vi "ArmControlManager.vi"(0 "Arm Rotate Manual Control":dbl, 1 "Arm Extend Manual Control":dbl, 2 "rotate sensor unit conversion (ticks/rad)":dbl, 3 "extend sensor unit coversion (ticks/in)":dbl, 4 "Arm Rotate Motion Profile":T1[](array[typedef]) {"Time (ms)" items=["TrajectoryDuration_0ms"=0, "TrajectoryDuration_5ms"=5, "TrajectoryDuration_10ms"=10, "TrajectoryDuration_20ms"=20, "TrajectoryDuration_30ms"=30, "TrajectoryDuration_40ms"=40, "TrajectoryDuration_50ms"=50, "TrajectoryDuration_100ms"=100]}, 5 "Arm Extend Motion Profile":T1[](array[typedef]) {"Time (ms)" items=["TrajectoryDuration_0ms"=0, "TrajectoryDuration_5ms"=5, "TrajectoryDuration_10ms"=10, "TrajectoryDuration_20ms"=20, "TrajectoryDuration_30ms"=30, "TrajectoryDuration_40ms"=40, "TrajectoryDuration_50ms"=50, "TrajectoryDuration_100ms"=100]}, 6 "ArmCompleteNotifier":refnum<notifier>, 8 "Arm Extend Motor DevRef":T4={"DeviceStatus"={"status"=FALSE, "code"=0, "source"=""}, "Type"=enum."PWM", "PWM"={"PWM Channel"=enum."PWM 1", "DeadBand"={"Name"="", "maxPositivePwm"=0, "minPositivePwm"=0, "centerPwm"=0, "maxNegativePwm"=0, "minNegativePwm"=0, "angularRange"=0}}, "CAN"={"Device Number"=0, "SetOutput VI Ref"=variant(enum8{"Percent VBus", "Current", "Speed", "Position", "Voltage"} enum."Percent VBus"), "GetOutput VI Ref"=variant(refnum<k1> refnum), "Enable VI Ref"=variant(dbl 12.0), "Disable VI Ref"=variant(enum8{"Percent VBus", "Speed", "Position", "Slave", "Unchanged / Invalid", "Voltage Compensation", "Current", "Motion Profile"} enum."Percent VBus"), "Data"=variant}, "Invert"=FALSE, "DIO PWM"={"PWM \"Enable\" Channel"=enum."Invalid", "DIOChannel"=enum."Invalid", "PWM Rate"=0.0}}, 9 "New Motion Profile":bool, 10 "Arm Rotate Motor DevRef":T4={"DeviceStatus"={"status"=FALSE, "code"=0, "source"=""}, "Type"=enum."PWM", "PWM"={"PWM Channel"=enum."PWM 1", "DeadBand"={"Name"="", "maxPositivePwm"=0, "minPositivePwm"=0, "centerPwm"=0, "maxNegativePwm"=0, "minNegativePwm"=0, "angularRange"=0}}, "CAN"={"Device Number"=0, "SetOutput VI Ref"=variant(enum8{"Percent VBus", "Current", "Speed", "Position", "Voltage"} enum."Percent VBus"), "GetOutput VI Ref"=variant(refnum<k1> refnum), "Enable VI Ref"=variant(dbl 12.0), "Disable VI Ref"=variant(enum8{"Percent VBus", "Speed", "Position", "Slave", "Unchanged / Invalid", "Voltage Compensation", "Current", "Motion Profile"} enum."Percent VBus"), "Data"=variant}, "Invert"=FALSE, "DIO PWM"={"PWM \"Enable\" Channel"=enum."Invalid", "DIOChannel"=enum."Invalid", "PWM Rate"=0.0}}) -> (14 "Arm Control State":T3)   [LabVIEW 2017]
uses:
  General/MotionProfiling/TypeDefs/TrajectoryPoint.ctl
  <vilib>/Rock Robotics/WPI/ThirdParty/Phoenix-LabVIEW/Motor Controller/Controls/CTRE_Phoenix_MotorControl_TrajectoryPointTimeDur.ctl
  General/MotionProfiling/TypeDefs/MotionProfileControlState.ctl
  <vilib>/Rock Robotics/WPI/MotorControl/WPI_MotorControlDeviceRef.ctl
  <vilib>/Rock Robotics/WPI/MotorControl/WPI_MotorControlType.ctl
  <vilib>/Rock Robotics/SystemInterfaces/DIO/FPGA_DIOPWMChannel.ctl
  <vilib>/Rock Robotics/WPI/PWM/WPI_PWMDeadband.ctl
  <vilib>/Rock Robotics/SystemInterfaces/DIO/FPGA_DIOChannel.ctl
  General/MotionProfiling/TypeDefs/MPSendState.ctl
  <vilib>/Rock Robotics/WPI/DriverStation/WPI_DriverStationRobotMode2.ctl
  ArgosLib/Signal Processing/TypeDefs/EdgeDetector_Type.ctl
  <vilib>/Rock Robotics/WPI/ThirdParty/Phoenix-LabVIEW/Motor Controller/Controls/CTRE_Phoenix_MotorControl_ControlMode.ctl
  Global_Var-RefNum/MotionProfileControlData.vi
  <vilib>/Rock Robotics/WPI/ThirdParty/Phoenix-LabVIEW/Motor Controller/Get/CTRE_Phoenix_MotorController_GetSelectedSensorData.vi
  <vilib>/Rock Robotics/WPI/ThirdParty/Phoenix-LabVIEW/Motor Controller/Get/CTRE_Phoenix_MotorController_GetVoltage.vi
  Global_Var-RefNum/LEDData.vi
  ArgosLib/ArgosLib.lvlib
panel:
  in  "MP State Timeout (ms)":u32
  in  "Tab Control":enum32{"I/O", "Calibration", "Status"}(tab)
  in  "ExtendErrorThresh (in)":dbl=3.0
  in  "RotateErrorThresh (rad)":dbl=0.1745
  in  "ClearMotionProfile":bool
  in  "StallDetectTime(ms)":u32=200
  in  "EnableStallDetection":bool
  out "Max Extend Speed (Sensor Units per 100 ms)":i32
  out "Max Rotate Speed (Sensor Units per 100 ms)":i32
  in  "Reset Rotate Max":bool
  in  "Reset Extend Max":bool
  in  "Reset Extend Sensor":bool
  in  "Reset Rotate Sensor":bool
  in  "Extend Position (in)":dbl=-44.0
  in  "Rotate Position (rad)":dbl=1.57
  out "MP Send State":T9
  out "Rotate":T10
  out "Extension":T10
  out "Rotate":T11
  out "Extension":T11
  out "ExtendFaults":T12
  out "RotateFaults":T12
  out "Arm Tracking":cluster{dbl[], dbl[]}[](graph)
  out "ArmRotateV":dbl(graph)
  out "ArmExtensionV":dbl(graph)
  out "ArmExtension":T11(graph)
  out "ArmRotation":T11(graph)
  # "10 degrees or 3 inches\nerror for 200ms will\ncancel motion"
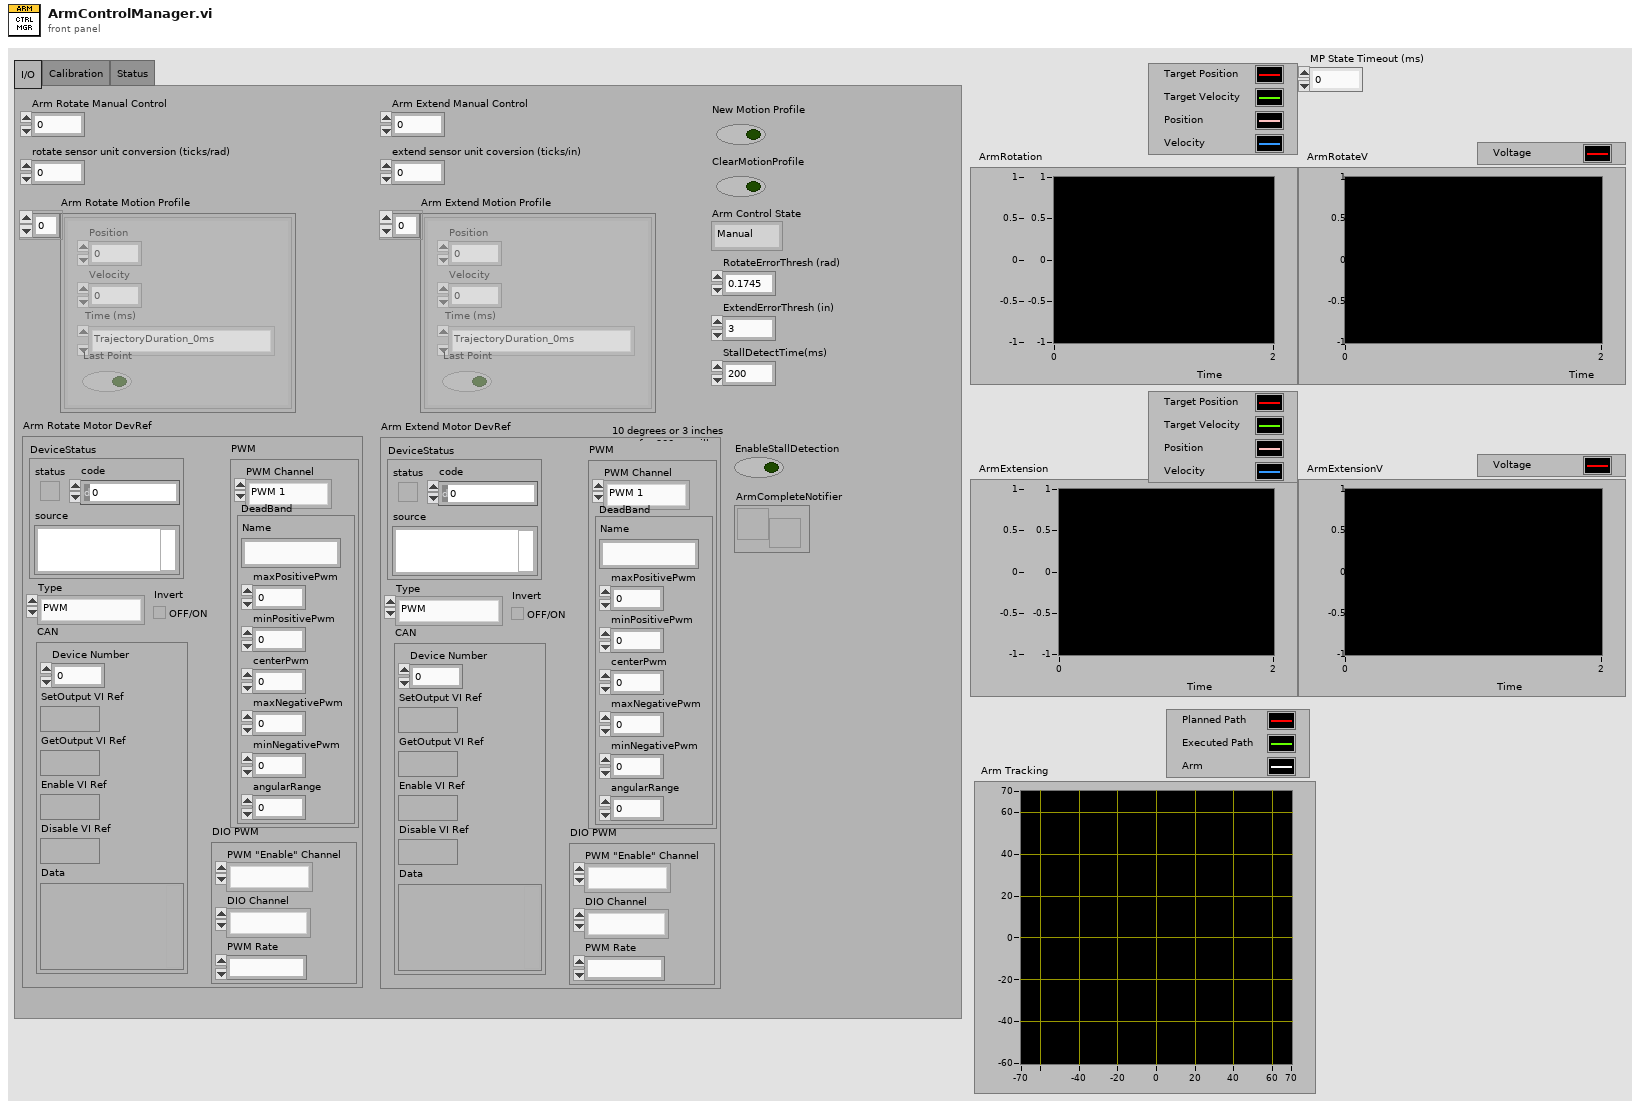
[diagram p1: front panel]
types:
  T1 = typedef "TrajectoryPoint.ctl" = cluster{"Position ":dbl, "Velocity ":dbl, "Time (ms)":T2, "Last Point":bool}
  T2 = typedef "CTRE_Phoenix_MotorControl_TrajectoryPointTimeDur.ctl" = i32
  T3 = typedef "MotionProfileControlState.ctl" = enum16{"Manual", "Auto_Idle", "Auto_Run"}
  T4 = typedef "WPI_MotorControlDeviceRef.ctl" = cluster{"DeviceStatus":errorcluster, "Type":T5, "PWM":cluster{"PWM Channel":T6, "DeadBand":T7}, "CAN":cluster{"Device Number":u8, "SetOutput VI Ref":variant, "GetOutput VI Ref":variant, "Enable VI Ref":variant, "Disable VI Ref":variant, "Data":variant}, "Invert":bool, "DIO PWM":cluster{"PWM \"Enable\" Channel":T6, "DIOChannel":T8, "PWM Rate":dbl}}
  T5 = typedef "WPI_MotorControlType.ctl" = enum16{"PWM", "CAN", "DIO PWM"}
  T6 = typedef "FPGA_DIOPWMChannel.ctl" = enum8{"PWM 0", "PWM 1", "PWM 2", "PWM 3", "PWM 4", "PWM 5", "PWM 6", "PWM 7", "PWM 8", "PWM 9", "PWM MXP 0", "PWM MXP 1", "PWM MXP 2", "PWM MXP 3", "PWM MXP 4", "PWM MXP 5", "PWM MXP 6", "PWM MXP 7", "PWM MXP 8", "PWM MXP 9", "Invalid"}
  T7 = typedef "WPI_PWMDeadband.ctl" = cluster{"Name":string, "maxPositivePwm":i32, "minPositivePwm":i32, "centerPwm":i32, "maxNegativePwm":i32, "minNegativePwm":i32, "angularRange":u16}
  T8 = typedef "FPGA_DIOChannel.ctl" = enum8{"DIO 0", "DIO 1", "DIO 2", "DIO 3", "DIO 4", "DIO 5", "DIO 6", "DIO 7", "DIO 8", "DIO 9", "DIO MXP 0", "DIO MXP 1", "DIO MXP 2", "DIO MXP 3", "DIO MXP 4", "DIO MXP 5", "DIO MXP 6", "DIO MXP 7", "DIO MXP 8", "DIO MXP 9", "DIO MXP 10", "DIO MXP 11", "DIO MXP 12", "DIO MXP 13", "DIO MXP 14", "DIO MXP 15", "SPI Port CS1", "SPI Port CS2", "SPI Port CS3", "SPI Port MISO", "SPI Port MOSI", "Invalid"}
  T9 = typedef "MPSendState.ctl" = enum16{"Disable", "Commit Points", "Enable", "Done", "Failed"}
  T10 = cluster{"Top Buffer Remaining":i32, "Top Buffer Count":i32, "Bottom Buffer Count":i32, "Has Underrun?":bool, "Is Underrun?":bool, "Active Point Valid?":bool, "Is Last?":bool, "Profile Slot Select 0":i32, "Output Enable":i32, "Time Duration (ms)":i32, "Profile Slot Select 1":i32}
  T11 = cluster{"Position (Sensor Units)":i32, "Velocity (Sensor Units per 100 ms)":i32, "Position (Raw Sensor Units)":i32, "Velocity (Raw Sensor Units per 100 ms)":i32}
  T12 = cluster{"Under Voltage":bool, "Forward Limit Switch":bool, "Reverse Limit Switch":bool, "Forward Soft Limit":bool, "Reverse Soft Limit":bool, "Hardware Failure":bool, "Reset During Enable":bool, "Sensor Overflow":bool, "Sensor Out of Phase":bool, "Hardware ESD Reset":bool, "Remote Loss of Signal":bool}
  T13 = typedef "WPI_DriverStationRobotMode2.ctl" = enum16{"Autonomous Disabled", "Autonomous Enabled", "Teleop Disabled", "Teleop Enabled", "Disconnected", "Finish", "Test Disabled", "Test Enabled", "Emergency Stopped"}
  T14 = typedef "ArgosLib.lvlib/EdgeDetector_Type.ctl" = enum16{"RisingEdge", "FallingEdge", "Both"}
  T15 = cluster{"Position (Sensor Units)":i32, "Velocity (Sensor Units per 100 ms)":i32, "Position (Raw Sensor Units)":i32, "Velocity (Raw Sensor Units per 100 ms)":i32}[]
  T16 = typedef "CTRE_Phoenix_MotorControl_ControlMode.ctl" = u16
  T17 = typedef "ArmMotionProfileControl.ctl" = cluster{"ControlMutex":T18, "Trajectory Points":T1[], "CurrentIndex":u32}
  T18 = typedef "Semaphore RefNum" = refnum<k1>
  T19 = cluster{"Position (Sensor Units)":i32, "Velocity (Sensor Units per 100 ms)":i32, "Position (Raw Sensor Units)":i32, i32}
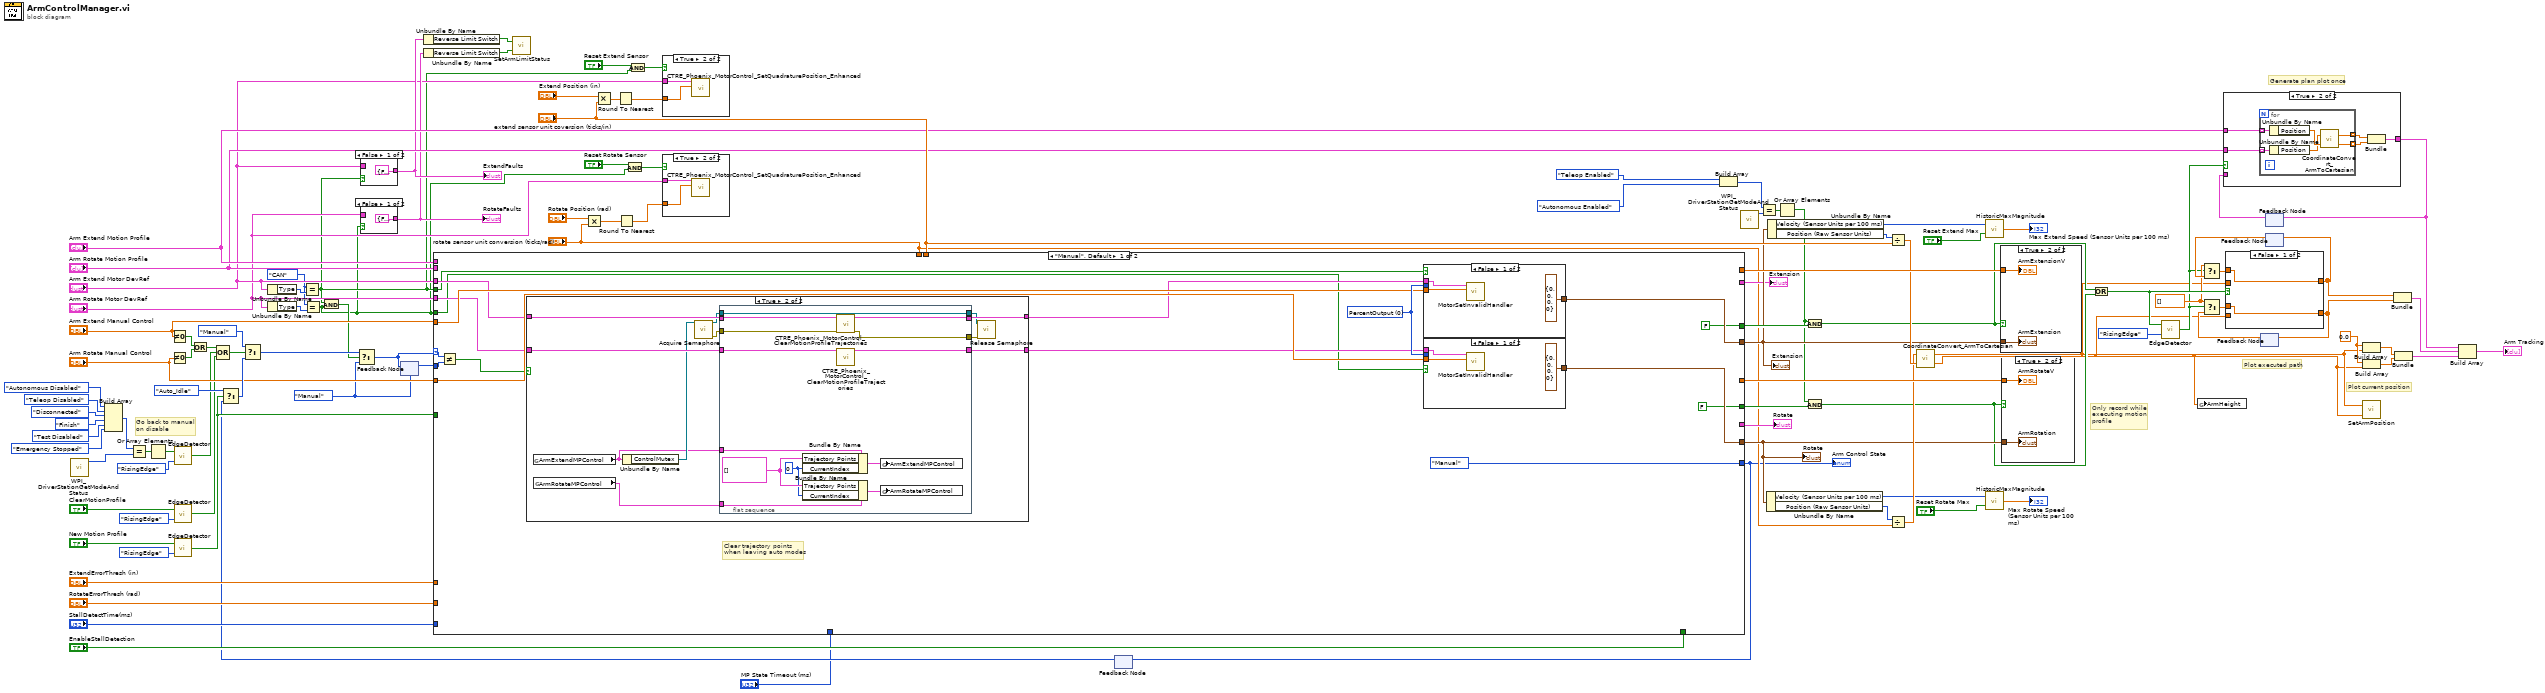
[diagram p0: block diagram]
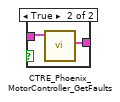
[diagram p2: hidden frame]
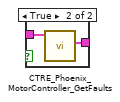
[diagram p3: hidden frame]
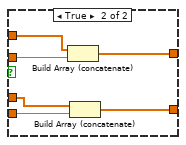
[diagram p5: hidden frame]
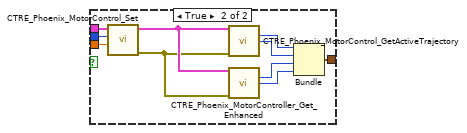
[diagram p10: hidden frame]
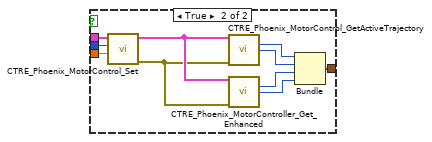
[diagram p11: hidden frame]
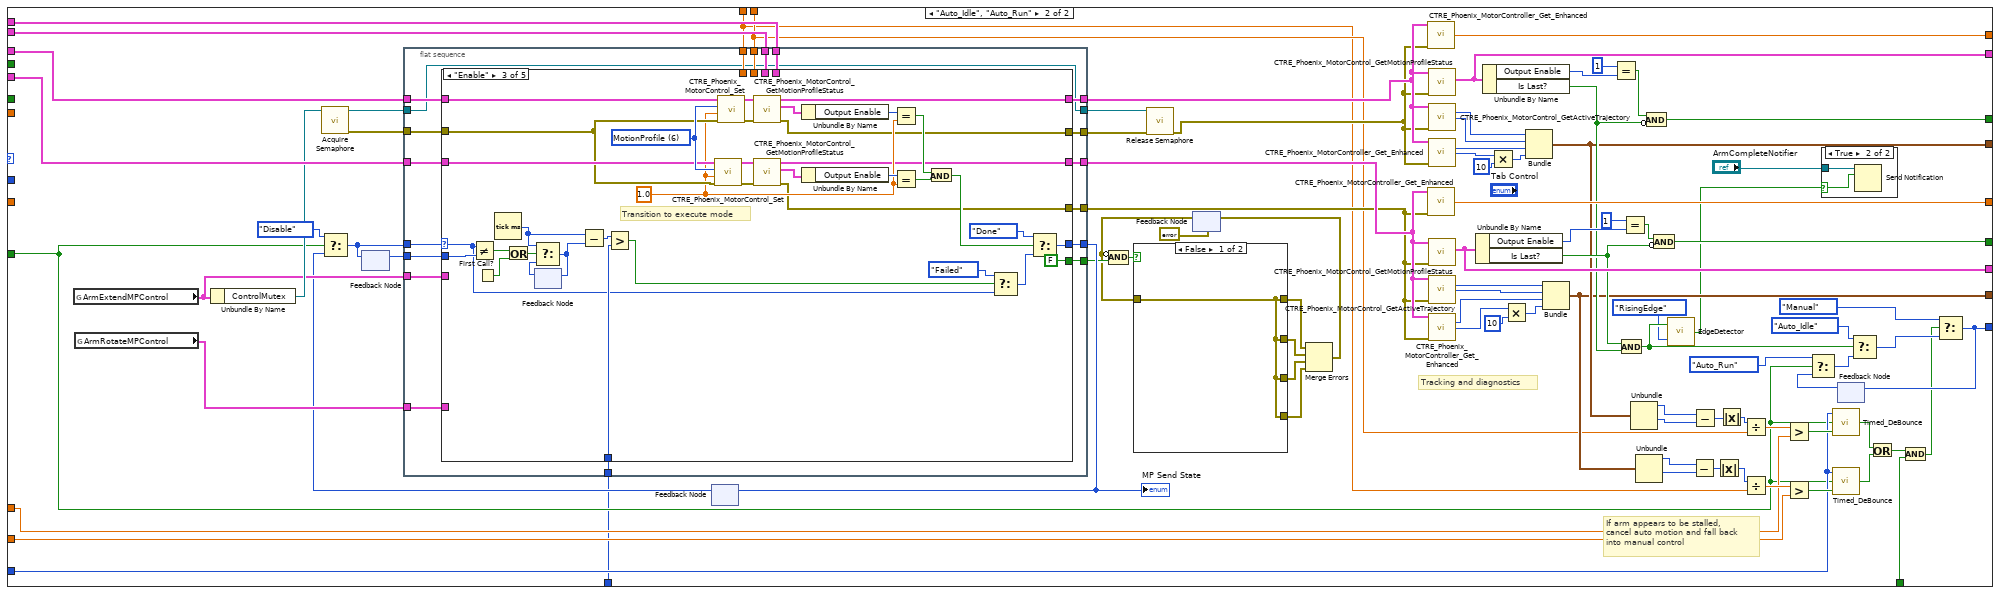
[diagram p13: hidden frame]
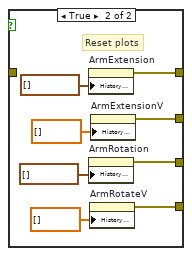
[diagram p15: hidden frame]
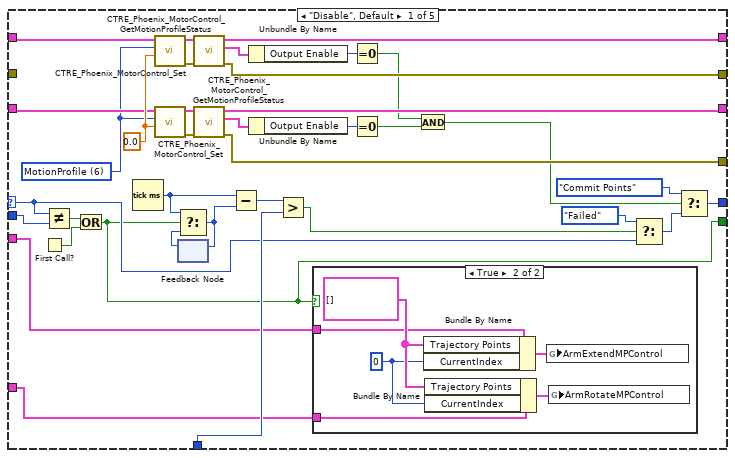
[diagram p16: hidden frame]
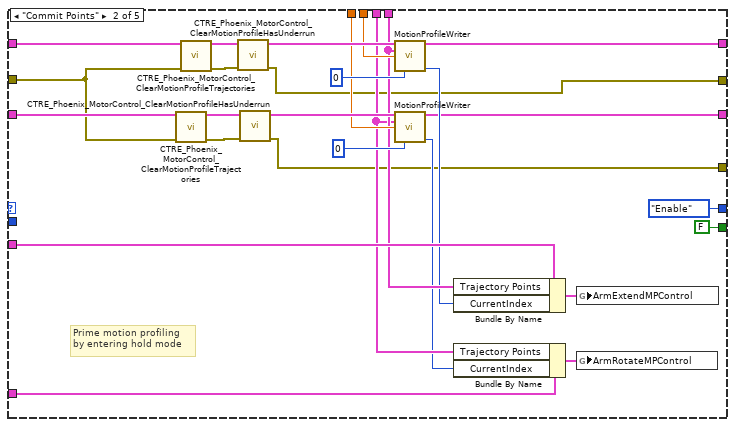
[diagram p18: hidden frame]
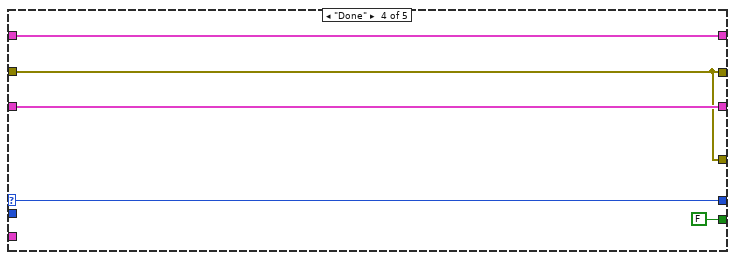
[diagram p19: hidden frame]
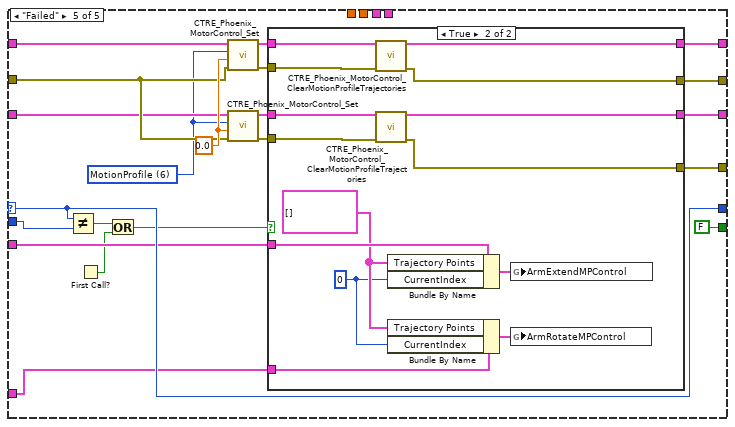
[diagram p20: hidden frame]
diagram:
  w7 = MotionProfileControlState."Manual" ("t")
  w10 = WPI_MotorControlType."CAN" ("x")
  w40 = dbl[] [] ("t")
  w74 = 0.0 ("element")
  # "Plot current position"
  # "Plot executed path"
  # "Generate plan plot once"
  # "Go back to manual\non disable"
  # "Only record while\nexecuting motion\nprofile"
  n1 = call <vilib>:"WPI_DriverStationGetModeAndStatus.vi"() -> ("Robot Mode"=w66:T13)  [unwired: 10 in, 1 out]
  n2 = Build Array(WPI_DriverStationRobotMode2."Autonomous Disabled" ("Robot Mode"), WPI_DriverStationRobotMode2."Teleop Disabled" ("Robot Mode"), WPI_DriverStationRobotMode2."Disconnected" ("Robot Mode"), WPI_DriverStationRobotMode2."Finish" ("Robot Mode"), WPI_DriverStationRobotMode2."Test Disabled" ("Robot Mode"), WPI_DriverStationRobotMode2."Emergency Stopped" ("Robot Mode")) -> (w67:T13[])
  n3 = Equal?(x=w67, y=w66) -> (x = y?=w65:bool[])
  n4 = Or Array Elements(Boolean array=w65) -> (logical OR=w64:bool)
  n5 = Not Equal To 0?(x="Arm Extend Manual Control") -> (x != 0?=w110:bool)
  n6 = Not Equal To 0?(x="Arm Rotate Manual Control") -> (x != 0?=w109:bool)
  n7 = call "EdgeDetector.vi"("DetectorType"=EdgeDetector_Type."RisingEdge", "Input"=w64) -> ("Edge"=w61:bool)
  n8 = call "EdgeDetector.vi"("DetectorType"=EdgeDetector_Type."RisingEdge", "Input"="ClearMotionProfile") -> ("Edge"=w62:bool)
  n9 = call "EdgeDetector.vi"("DetectorType"=EdgeDetector_Type."RisingEdge", "Input"="New Motion Profile") -> ("Edge"=w103:bool)
  n10 = Or(x=w110, y=w109) -> (x .or. y?=w92:bool)
  n11 = Compound Arithmetic op=OR(w92, w61, w62) -> (w93:bool)
  n12 = Unbundle By Name("Arm Extend Motor DevRef") -> ("Type"=w12:T5)
  n13 = Unbundle By Name("Arm Rotate Motor DevRef") -> ("Type"=w11:T5)
  n14 = Equal?(x=w10, y=w12) -> (x = y?=w2:bool)
  n15 = Equal?(x=w10, y=w11) -> (x = y?=w1:bool)
  n16 = And(x=w2, y=w1) -> (x .and. y?=w6:bool)
  n17 = case shown="False" w2 {
    tunnel: [T12 {"Under Voltage"=FALSE, "Forward Limit Switch"=FALSE, "Reverse Limit Switch"=FALSE, "Forward Soft Limit"=FALSE, "Reverse Soft Limit"=FALSE, "Hardware Failure"=FALSE, "Reset During Enable"=FALSE, "Sensor Overflow"=FALSE, "Sensor Out of Phase"=FALSE, "Hardware ESD Reset"=FALSE, "Remote Loss of Signal"=FALSE} ("Faults") w113] -> w18
    tunnel: "Arm Extend Motor DevRef" -> [_ w112]
    frame False {
    }
    frame True {
      n18 = call <vilib>:"CTRE_Phoenix_MotorController_GetFaults.vi"("PhoenixMotorControlDevRef"=w112) -> ("Faults"=w113:T12)  [unwired: 8 in, 2 out]
    }
  }
  "ExtendFaults" <- w18
  n19 = case shown="False" w1 {
    tunnel: [T12 {"Under Voltage"=FALSE, "Forward Limit Switch"=FALSE, "Reverse Limit Switch"=FALSE, "Forward Soft Limit"=FALSE, "Reverse Soft Limit"=FALSE, "Hardware Failure"=FALSE, "Reset During Enable"=FALSE, "Sensor Overflow"=FALSE, "Sensor Out of Phase"=FALSE, "Hardware ESD Reset"=FALSE, "Remote Loss of Signal"=FALSE} ("Faults") w116] -> w17
    tunnel: "Arm Rotate Motor DevRef" -> [_ w115]
    frame False {
    }
    frame True {
      n20 = call <vilib>:"CTRE_Phoenix_MotorController_GetFaults.vi"("PhoenixMotorControlDevRef"=w115) -> ("Faults"=w116:T12)  [unwired: 8 in, 2 out]
    }
  }
  "RotateFaults" <- w17
  n21 = feedback #1(w7) -> (w23:T3)
  n22 = Unbundle By Name(w18) -> ("Reverse Limit Switch"=w16:bool)
  n23 = Unbundle By Name(w17) -> ("Reverse Limit Switch"=w15:bool)
  n24 = call "SetArmLimitStatus.vi"("ArmRotateLimit"=w15, "ArmExtendLimit"=w16) -> ()  [unwired: 1 in]
  n25 = Multiply(x="Rotate Position (rad)", y="rotate sensor unit conversion (ticks/rad)") -> (x*y=w78:dbl)
  n26 = Multiply(x="Extend Position (in)", y="extend sensor unit coversion (ticks/in)") -> (x*y=w81:dbl)
  n27 = Round To Nearest(number=w81) -> (nearest integer value=w80:dbl)
  n28 = Round To Nearest(number=w78) -> (nearest integer value=w77:dbl)
  n29 = And(x="Reset Rotate Sensor", y=w1) -> (x .and. y?=w4:bool)
  n30 = And(x="Reset Extend Sensor", y=w2) -> (x .and. y?=w5:bool)
  n31 = case shown="True" w5 {
    tunnel: "Arm Extend Motor DevRef" -> [_ w118]
    tunnel: w80 -> [_ w117]
    frame False {
    }
    frame True {
      n32 = call <vilib>:"CTRE_Phoenix_MotorControl_SetQuadraturePosition_Enhanced.vi"("New Position"=w117, "PhoenixMotorControlDevRef"=w118) -> ()  [unwired: 8 in, 2 out]
    }
  }
  n33 = case shown="True" w4 {
    tunnel: "Arm Rotate Motor DevRef" -> [_ w120]
    tunnel: w77 -> [_ w119]
    frame False {
    }
    frame True {
      n34 = call <vilib>:"CTRE_Phoenix_MotorControl_SetQuadraturePosition_Enhanced.vi"("New Position"=w119, "PhoenixMotorControlDevRef"=w120) -> ()  [unwired: 8 in, 2 out]
    }
  }
  n35 = feedback #2() -> (w22:T3)  [unwired: 1 in]
  n36 = Select(t=MotionProfileControlState."Auto_Idle", s=w103, f=w22) -> (s? t:f=w107:T3)
  n37 = Select(t=MotionProfileControlState."Manual" ("Arm Control State"), s=w93, f=w107) -> (s? t:f=w9:T3)
  n38 = Select(t=w9, s=w6, f=w7) -> (s? t:f=w8:T3)
  n39 = feedback-in #1(w8) -> ()
  n40 = case shown="\"Manual\", Default" w8 {
    selector: w8 -> [w135 _]
    tunnel: "Arm Extend Motor DevRef" -> [w127 w239]
    tunnel: "Arm Rotate Motor DevRef" -> [w126 w238]
    tunnel: "Arm Extend Manual Control" -> [w128 _]
    tunnel: "Arm Rotate Manual Control" -> [w136 _]
    tunnel: w23 -> [w134 _]
    tunnel: w103 -> [_ w209]
    tunnel: "Arm Extend Motion Profile" -> [_ w241]
    tunnel: "Arm Rotate Motion Profile" -> [_ w240]
    tunnel: [MotionProfileControlState."Manual" ("Arm Control State") w244] -> w24
    tunnel: [w132 w229] -> w76
    tunnel: [w131 w228] -> w75
    tunnel: [FALSE w271] -> w96
    tunnel: [FALSE w267] -> w98
    tunnel: [_ w260] -> w95
    tunnel: [_ w259] -> w94
    tunnel: "extend sensor unit coversion (ticks/in)" -> [_ w219]
    tunnel: "rotate sensor unit conversion (ticks/rad)" -> [_ w217]
    tunnel: [_ w255] -> w54
    tunnel: [_ w254] -> w53
    tunnel: "ExtendErrorThresh (in)" -> [_ w250]
    tunnel: "RotateErrorThresh (rad)" -> [_ w251]
    tunnel: "StallDetectTime(ms)" -> [_ w247]
    tunnel: "EnableStallDetection" -> [_ w221]
    tunnel: "MP State Timeout (ms)" -> [_ w204]
    tunnel: w2 -> [w122 _]
    tunnel: w1 -> [w121 _]
    frame "Manual", Default {
      w137 = T16 0 items=["PercentOutput"=0, "Position"=1, "Velocity"=2, "Current"=3, "Follower"=5, "MotionProfile"=6, "MotionMagic"=7, "MotionMagicArc"=8, "MotionProfileArc"=10, "Disabled"=15] ("Control Mode")
      # "Clear trajectory points\nwhen leaving auto modes"
      n41 = Not Equal?(x=w135, y=w134) -> (x != y?=w123:bool)
      n42 = case shown="True" w123 {
        tunnel: w127 -> [w165 w176]
        tunnel: [w165 w175] -> w125
        tunnel: w126 -> [w164 w174]
        tunnel: [w164 w173] -> w124
        frame False {
        }
        frame True {
          n43 = global read "MotionProfileControlData.vi" "ArmExtendMPControl"() -> (w169:T17)
          n44 = global read "MotionProfileControlData.vi" "ArmRotateMPControl"() -> (w168:T17)
          n45 = Unbundle By Name(w169) -> ("ControlMutex"=w171:T18)
          n46 = call <vilib>:"Acquire Semaphore.vi"("semaphore"=w171) -> ("error out"=w172:errorcluster, "semaphore out"=w167:T18)  [unwired: 4 in, 1 out]
          n47 = flat-sequence {
            tunnel: w176 -> [w189]
            tunnel: [w188] -> w175
            tunnel: w174 -> [w187]
            tunnel: [w186] -> w173
            tunnel: w172 -> [w185]
            tunnel: [w184] -> w170
            tunnel: w169 -> [w183]
            tunnel: w168 -> [w182]
            tunnel: w167 -> [w177]
            tunnel: [w177] -> w166
            frame #0 {
              w180 = u32 0 ("CurrentIndex")
              w181 = T1[] [] ("Trajectory Points")
              n48 = Bundle By Name(cluster=w183, "Trajectory Points"=w181, "CurrentIndex"=w180) -> (w178:T17)
              n49 = Bundle By Name(cluster=w182, "Trajectory Points"=w181, "CurrentIndex"=w180) -> (w179:T17)
              n50 = call <vilib>:"CTRE_Phoenix_MotorControl_ClearMotionProfileTrajectories.vi"("PhoenixMotorControlDevRef"=w189, "error in"=w185) -> ("PhoenixMotorControlDevRef"=w188:T4, "error out"=w184:errorcluster)  [unwired: 12 in]
              n51 = call <vilib>:"CTRE_Phoenix_MotorControl_ClearMotionProfileTrajectories.vi"("PhoenixMotorControlDevRef"=w187) -> ("PhoenixMotorControlDevRef"=w186:T4)  [unwired: 13 in, 1 out]
              n52 = global write "MotionProfileControlData.vi" "ArmExtendMPControl"(w178) -> ()
              n53 = global write "MotionProfileControlData.vi" "ArmRotateMPControl"(w179) -> ()
            }
          }
          n54 = call <vilib>:"Release Semaphore.vi"("error in (no error)"=w170, "semaphore"=w166) -> ()  [unwired: 4 in, 2 out]
        }
      }
      n55 = case shown="False" w122 {
        tunnel: w137 -> [_ w163]
        tunnel: [T11 {"Position (Sensor Units)"=0, "Velocity (Sensor Units per 100 ms)"=0, "Position (Raw Sensor Units)"=0, "Velocity (Raw Sensor Units per 100 ms)"=0} w162] -> w132
        tunnel: w128 -> [w152 w155]
        tunnel: w125 -> [w153 w154]
        frame False {
          n56 = call "MotorSetInvalidHandler.vi"("Output"=w152, "MotorControlDevRef"=w153) -> ()  [unwired: 7 in, 3 out]
        }
        frame True {
          n57 = call <vilib>:"CTRE_Phoenix_MotorControl_Set.vi"("Output"=w155, "Control Mode"=w163, "PhoenixMotorControlDevRef"=w154) -> ("error out"=w160:errorcluster, "PhoenixMotorControlDevRef"=w161:T4)  [unwired: 7 in]
          n58 = call <vilib>:"CTRE_Phoenix_MotorControl_GetActiveTrajectory.vi"("PhoenixMotorControlDevRef"=w161, "error in"=w160) -> ("Position (Sensor Units)"=w159:i32, "Velocity (Sensor Units per 100 ms)"=w158:i32)  [unwired: 9 in, 3 out]
          n59 = call-poly <vilib>:"CTRE_Phoenix_MotorController_Get_Enhanced.vi"("PhoenixMotorControlDevRef"=w161, "error in"=w160) -> ("Position (Raw Sensor Units)"=w157:i32, "Velocity (Raw Sensor Units per 100 ms)"=w156:i32)  [unwired: 10 in, 2 out]
          n60 = Bundle("Position (Sensor Units)"=w159, "Velocity (Sensor Units per 100 ms)"=w158, "Position (Raw Sensor Units)"=w157, "Velocity (Raw Sensor Units per 100 ms)"=w156) -> (w162:T11)  [unwired: 1 in]
        }
      }
      n61 = case shown="False" w121 {
        tunnel: w137 -> [_ w150]
        tunnel: w136 -> [w139 w149]
        tunnel: [T11 {"Position (Sensor Units)"=0, "Velocity (Sensor Units per 100 ms)"=0, "Position (Raw Sensor Units)"=0, "Velocity (Raw Sensor Units per 100 ms)"=0} w142] -> w131
        tunnel: w124 -> [w140 w141]
        frame False {
          n62 = call "MotorSetInvalidHandler.vi"("Output"=w139, "MotorControlDevRef"=w140) -> ()  [unwired: 7 in, 3 out]
        }
        frame True {
          n63 = call <vilib>:"CTRE_Phoenix_MotorControl_Set.vi"("Output"=w149, "Control Mode"=w150, "PhoenixMotorControlDevRef"=w141) -> ("error out"=w147:errorcluster, "PhoenixMotorControlDevRef"=w148:T4)  [unwired: 7 in]
          n64 = call <vilib>:"CTRE_Phoenix_MotorControl_GetActiveTrajectory.vi"("PhoenixMotorControlDevRef"=w148, "error in"=w147) -> ("Position (Sensor Units)"=w146:i32, "Velocity (Sensor Units per 100 ms)"=w145:i32)  [unwired: 9 in, 3 out]
          n65 = call-poly <vilib>:"CTRE_Phoenix_MotorController_Get_Enhanced.vi"("PhoenixMotorControlDevRef"=w148, "error in"=w147) -> ("Position (Raw Sensor Units)"=w144:i32, "Velocity (Raw Sensor Units per 100 ms)"=w143:i32)  [unwired: 10 in, 2 out]
          n66 = Bundle("Position (Sensor Units)"=w146, "Velocity (Sensor Units per 100 ms)"=w145, "Position (Raw Sensor Units)"=w144, "Velocity (Raw Sensor Units per 100 ms)"=w143) -> (w142:T11)  [unwired: 1 in]
        }
      }
    }
    frame "Auto_Idle", "Auto_Run" {
      # "If arm appears to be stalled,\ncancel auto motion and fall back\ninto manual control"
      # "Tracking and diagnostics"
      n67 = global read "MotionProfileControlData.vi" "ArmExtendMPControl"() -> (w214:T17)
      n68 = global read "MotionProfileControlData.vi" "ArmRotateMPControl"() -> (w213:T17)
      n69 = Unbundle By Name(w214) -> ("ControlMutex"=w215:T18)
      n70 = call <vilib>:"Acquire Semaphore.vi"("semaphore"=w215) -> ("error out"=w216:errorcluster, "semaphore out"=w211:T18)  [unwired: 4 in, 1 out]
      n71 = feedback #3() -> (w205:T9)  [unwired: 1 in]
      n72 = flat-sequence {
        tunnel: w239 -> [w311]
        tunnel: w238 -> [w310]
        tunnel: w216 -> [w309]
        tunnel: w219 -> [w308]
        tunnel: w217 -> [w307]
        tunnel: [w306] -> w237
        tunnel: [w305] -> w235
        tunnel: w214 -> [w304]
        tunnel: w213 -> [w303]
        tunnel: w241 -> [w302]
        tunnel: w240 -> [w301]
        tunnel: [w300] -> w212
        tunnel: [w299] -> w234
        tunnel: w211 -> [w298]
        tunnel: [w298] -> w210
        tunnel: w206 -> [w297]
        tunnel: [w296] -> w203
        tunnel: w205 -> [w295]
        tunnel: w204 -> [w294]
        tunnel: [w293] -> w193
        frame #0 {
          n73 = case shown="\"Enable\"" w297 {
            selector: w297 -> [w315 _ w385 w418 w437]
            tunnel: w311 -> [w342 w362 w415 w421 w441]
            tunnel: w310 -> [w341 w361 w414 w420 w439]
            tunnel: w309 -> [_ w360 w413 w419 w440]
            tunnel: w308 -> [_ w372 _ _ _]
            tunnel: w307 -> [_ w371 _ _ _]
            tunnel: [w334 w358 w389 w421 w430] -> w306
            tunnel: [w335 w359 w387 w420 w428] -> w305
            tunnel: w304 -> [w318 w370 _ _ w425]
            tunnel: w303 -> [w317 w369 _ _ w426]
            tunnel: w302 -> [_ w368 _ _ _]
            tunnel: w301 -> [_ w367 _ _ _]
            tunnel: [w333 w356 w388 w419 w429] -> w300
            tunnel: [w332 w357 w386 w419 w427] -> w299
            tunnel: [w325 MPSendState."Enable" ("MP Send State") w403 w418 w437] -> w296
            tunnel: w295 -> [w324 _ w408 _ w436]
            tunnel: w294 -> [w319 _ w407 _ _]
            tunnel: [w313 FALSE FALSE FALSE FALSE] -> w293
            frame "Disable", Default {
              w347 = 0.0 ("Output")
              w340 = T16 6 items=["PercentOutput"=0, "Position"=1, "Velocity"=2, "Current"=3, "Follower"=5, "MotionProfile"=6, "MotionMagic"=7, "MotionMagicArc"=8, "MotionProfileArc"=10, "Disabled"=15] ("Control Mode")
              n74 = First Call?() -> (First Call?: T/F=w312:bool)
              n75 = Not Equal?(x=w315, y=w324) -> (x != y?=w314:bool)
              n76 = Or(x=w314, y=w312) -> (x .or. y?=w313:bool)
              n77 = Tick Count (ms)() -> (millisecond timer value=w322:u32)
              n78 = call <vilib>:"CTRE_Phoenix_MotorControl_Set.vi"("Output"=w347, "Control Mode"=w340, "PhoenixMotorControlDevRef"=w342) -> ("error out"=w345:errorcluster, "PhoenixMotorControlDevRef"=w346:T4)  [unwired: 7 in]
              n79 = call <vilib>:"CTRE_Phoenix_MotorControl_Set.vi"("Output"=w347, "Control Mode"=w340, "PhoenixMotorControlDevRef"=w341) -> ("error out"=w344:errorcluster, "PhoenixMotorControlDevRef"=w343:T4)  [unwired: 7 in]
              n80 = feedback #4() -> (w323:u32)  [unwired: 1 in]
              n81 = Select(t=w322, s=w313, f=w323) -> (s? t:f=w321:u32)
              n82 = feedback-in #4(w321) -> ()
              n83 = call <vilib>:"CTRE_Phoenix_MotorControl_GetMotionProfileStatus.vi"("error in"=w345, "PhoenixMotorControlDevRef"=w346) -> ("error out"=w333:errorcluster, "Motion Profile Status"=w339:T10, "PhoenixMotorControlDevRef"=w334:T4)  [unwired: 7 in]
              n84 = call <vilib>:"CTRE_Phoenix_MotorControl_GetMotionProfileStatus.vi"("error in"=w344, "PhoenixMotorControlDevRef"=w343) -> ("error out"=w332:errorcluster, "Motion Profile Status"=w338:T10, "PhoenixMotorControlDevRef"=w335:T4)  [unwired: 7 in]
              n85 = Subtract(x=w322, y=w321) -> (x-y=w320:u32)
              n86 = Unbundle By Name(w339) -> ("Output Enable"=w337:i32)
              n87 = Unbundle By Name(w338) -> ("Output Enable"=w336:i32)
              n88 = Greater?(x=w320, y=w319) -> (0:w316:bool)
              n89 = case shown="True" w313 {
                tunnel: w318 -> [_ w349]
                tunnel: w317 -> [_ w348]
                frame False {
                }
                frame True {
                  w350 = u32 0 ("CurrentIndex")
                  w351 = T1[] [] ("Trajectory Points")
                  n90 = Bundle By Name(cluster=w349, "Trajectory Points"=w351, "CurrentIndex"=w350) -> (w353:T17)
                  n91 = Bundle By Name(cluster=w348, "Trajectory Points"=w351, "CurrentIndex"=w350) -> (w352:T17)
                  n92 = global write "MotionProfileControlData.vi" "ArmExtendMPControl"(w353) -> ()
                  n93 = global write "MotionProfileControlData.vi" "ArmRotateMPControl"(w352) -> ()
                }
              }
              n94 = Equal To 0?(x=w337) -> (x = 0?=w331:bool)
              n95 = Equal To 0?(x=w336) -> (x = 0?=w330:bool)
              n96 = And(x=w331, y=w330) -> (x .and. y?=w329:bool)
              n97 = Select(t=MPSendState."Failed", s=w316, f=w315) -> (s? t:f=w328:T9)
              n98 = Select(t=MPSendState."Commit Points", s=w329, f=w328) -> (s? t:f=w325:T9)
            }
            frame "Commit Points" {
              # "Prime motion profiling\nby entering hold mode"
              n99 = call <vilib>:"CTRE_Phoenix_MotorControl_ClearMotionProfileTrajectories.vi"("PhoenixMotorControlDevRef"=w361, "error in"=w360) -> ("PhoenixMotorControlDevRef"=w380:T4, "error out"=w379:errorcluster)  [unwired: 12 in]
              n100 = call <vilib>:"CTRE_Phoenix_MotorControl_ClearMotionProfileTrajectories.vi"("PhoenixMotorControlDevRef"=w362, "error in"=w360) -> ("PhoenixMotorControlDevRef"=w378:T4, "error out"=w377:errorcluster)  [unwired: 12 in]
              n101 = call <vilib>:"CTRE_Phoenix_MotorControl_ClearMotionProfileHasUnderrun.vi"("error in"=w377, "PhoenixMotorControlDevRef"=w378) -> ("error out"=w356:errorcluster, "PhoenixMotorControlDevRef"=w376:T4)  [unwired: 8 in]
              n102 = call <vilib>:"CTRE_Phoenix_MotorControl_ClearMotionProfileHasUnderrun.vi"("error in"=w379, "PhoenixMotorControlDevRef"=w380) -> ("error out"=w357:errorcluster, "PhoenixMotorControlDevRef"=w375:T4)  [unwired: 8 in]
              n103 = call "MotionProfileWriter.vi"("PhoenixMotorControlDevRef"=w376, "Trajectory Points"=w368, "Sensor unit conversion"=w372, "startIndex"=0) -> ("PhoenixMotorControlDevRef Out"=w358:T4, "endIndex"=w366:i32)  [unwired: 10 in]
              n104 = call "MotionProfileWriter.vi"("PhoenixMotorControlDevRef"=w375, "Trajectory Points"=w367, "Sensor unit conversion"=w371, "startIndex"=0) -> ("PhoenixMotorControlDevRef Out"=w359:T4, "endIndex"=w365:i32)  [unwired: 10 in]
              n105 = Bundle By Name(cluster=w370, "Trajectory Points"=w368, "CurrentIndex"=w366) -> (w364:T17)
              n106 = Bundle By Name(cluster=w369, "Trajectory Points"=w367, "CurrentIndex"=w365) -> (w363:T17)
              n107 = global write "MotionProfileControlData.vi" "ArmExtendMPControl"(w364) -> ()
              n108 = global write "MotionProfileControlData.vi" "ArmRotateMPControl"(w363) -> ()
            }
            frame "Enable" {
              w391 = 1.0 ("Output")
              w416 = T16 6 items=["PercentOutput"=0, "Position"=1, "Velocity"=2, "Current"=3, "Follower"=5, "MotionProfile"=6, "MotionMagic"=7, "MotionMagicArc"=8, "MotionProfileArc"=10, "Disabled"=15] ("Control Mode")
              # "Transition to execute mode"
              n109 = Not Equal?(x=w385, y=w408) -> (x != y?=w382:bool)
              n110 = First Call?() -> (First Call?: T/F=w381:bool)
              n111 = Tick Count (ms)() -> (millisecond timer value=w411:u32)
              n112 = Or(x=w382, y=w381) -> (x .or. y?=w383:bool)
              n113 = feedback #5() -> (w412:u32)  [unwired: 1 in]
              n114 = Select(t=w411, s=w383, f=w412) -> (s? t:f=w410:u32)
              n115 = feedback-in #5(w410) -> ()
              n116 = Subtract(x=w411, y=w410) -> (x-y=w409:u32)
              n117 = Greater?(x=w409, y=w407) -> (0:w402:bool)
              n118 = call <vilib>:"CTRE_Phoenix_MotorControl_Set.vi"("error in (no error)"=w413, "Output"=w391, "Control Mode"=w416, "PhoenixMotorControlDevRef"=w414) -> ("error out"=w396:errorcluster, "PhoenixMotorControlDevRef"=w397:T4)  [unwired: 6 in]
              n119 = call <vilib>:"CTRE_Phoenix_MotorControl_Set.vi"("error in (no error)"=w413, "Output"=w391, "Control Mode"=w416, "PhoenixMotorControlDevRef"=w415) -> ("error out"=w394:errorcluster, "PhoenixMotorControlDevRef"=w395:T4)  [unwired: 6 in]
              n120 = call <vilib>:"CTRE_Phoenix_MotorControl_GetMotionProfileStatus.vi"("error in"=w394, "PhoenixMotorControlDevRef"=w395) -> ("error out"=w388:errorcluster, "Motion Profile Status"=w401:T10, "PhoenixMotorControlDevRef"=w389:T4)  [unwired: 7 in]
              n121 = call <vilib>:"CTRE_Phoenix_MotorControl_GetMotionProfileStatus.vi"("error in"=w396, "PhoenixMotorControlDevRef"=w397) -> ("error out"=w386:errorcluster, "Motion Profile Status"=w400:T10, "PhoenixMotorControlDevRef"=w387:T4)  [unwired: 7 in]
              n122 = Unbundle By Name(w401) -> ("Output Enable"=w393:i32)
              n123 = Unbundle By Name(w400) -> ("Output Enable"=w392:i32)
              n124 = Equal?(x=w393, y=w391) -> (x = y?=w399:bool)
              n125 = Equal?(x=w392, y=w391) -> (x = y?=w398:bool)
              n126 = And(x=w399, y=w398) -> (x .and. y?=w390:bool)
              n127 = Select(t=MPSendState."Failed", s=w402, f=w385) -> (s? t:f=w406:T9)
              n128 = Select(t=MPSendState."Done", s=w390, f=w406) -> (s? t:f=w403:T9)
            }
            frame "Done" {
            }
            frame "Failed" {
              w442 = 0.0 ("Output")
              w438 = T16 6 items=["PercentOutput"=0, "Position"=1, "Velocity"=2, "Current"=3, "Follower"=5, "MotionProfile"=6, "MotionMagic"=7, "MotionMagicArc"=8, "MotionProfileArc"=10, "Disabled"=15] ("Control Mode")
              n129 = Not Equal?(x=w437, y=w436) -> (x != y?=w435:bool)
              n130 = First Call?() -> (First Call?: T/F=w422:bool)
              n131 = Or(x=w435, y=w422) -> (x .or. y?=w423:bool)
              n132 = call <vilib>:"CTRE_Phoenix_MotorControl_Set.vi"("error in (no error)"=w440, "Output"=w442, "Control Mode"=w438, "PhoenixMotorControlDevRef"=w441) -> ("error out"=w432:errorcluster, "PhoenixMotorControlDevRef"=w434:T4)  [unwired: 6 in]
              n133 = call <vilib>:"CTRE_Phoenix_MotorControl_Set.vi"("error in (no error)"=w440, "Output"=w442, "Control Mode"=w438, "PhoenixMotorControlDevRef"=w439) -> ("error out"=w431:errorcluster, "PhoenixMotorControlDevRef"=w433:T4)  [unwired: 6 in]
              n134 = case shown="True" w423 {
                tunnel: w434 -> [w446 w460]
                tunnel: w433 -> [w444 w458]
                tunnel: w432 -> [w445 w459]
                tunnel: w431 -> [w443 w457]
                tunnel: [w446 w456] -> w430
                tunnel: [w445 w455] -> w429
                tunnel: [w444 w454] -> w428
                tunnel: [w443 w453] -> w427
                tunnel: w426 -> [_ w450]
                tunnel: w425 -> [_ w449]
                frame False {
                }
                frame True {
                  w447 = u32 0 ("CurrentIndex")
                  w448 = T1[] [] ("Trajectory Points")
                  n135 = call <vilib>:"CTRE_Phoenix_MotorControl_ClearMotionProfileTrajectories.vi"("PhoenixMotorControlDevRef"=w460, "error in"=w459) -> ("PhoenixMotorControlDevRef"=w456:T4, "error out"=w455:errorcluster)  [unwired: 12 in]
                  n136 = call <vilib>:"CTRE_Phoenix_MotorControl_ClearMotionProfileTrajectories.vi"("PhoenixMotorControlDevRef"=w458, "error in"=w457) -> ("PhoenixMotorControlDevRef"=w454:T4, "error out"=w453:errorcluster)  [unwired: 12 in]
                  n137 = Bundle By Name(cluster=w449, "Trajectory Points"=w448, "CurrentIndex"=w447) -> (w452:T17)
                  n138 = Bundle By Name(cluster=w450, "Trajectory Points"=w448, "CurrentIndex"=w447) -> (w451:T17)
                  n139 = global write "MotionProfileControlData.vi" "ArmExtendMPControl"(w452) -> ()
                  n140 = global write "MotionProfileControlData.vi" "ArmRotateMPControl"(w451) -> ()
                }
              }
            }
          }
        }
      }
      n141 = feedback-in #6(w203) -> ()
      n142 = feedback #6() -> (w207:T9)  [unwired: 1 in]
      n143 = Select(t=MPSendState."Disable" ("MP Send State"), s=w209, f=w207) -> (s? t:f=w206:T9)
      n144 = feedback-in #3(w206) -> ()
      n145 = call <vilib>:"Release Semaphore.vi"("error in (no error)"=w212, "semaphore"=w210) -> ("error out"=w236:errorcluster)  [unwired: 4 in, 1 out]
      n146 = feedback #7(errorcluster {"status"=FALSE, "code"=0, "source"=""} ("error IO")) -> (w190:errorcluster)
      n147 = Compound Arithmetic op=AND(invert w190, w193) -> (w192:bool)
      n148 = case shown="False" w192 {
        tunnel: [w284 w288] -> w198
        tunnel: [w284 w287] -> w197
        tunnel: [w284 w286] -> w196
        tunnel: [w284 w285] -> w195
        tunnel: w190 -> [w284 _]
        frame False {
        }
        frame True {
          # "Reset plots"
          n149 = property on="ArmExtension" class="WFChart (strict)"("History Data"=T15 []) -> (error out=w288:errorcluster)  [unwired: 2 in, 1 out]
          n150 = property on="ArmRotation" class="WFChart (strict)"("History Data"=T15 []) -> (error out=w286:errorcluster)  [unwired: 2 in, 1 out]
          n151 = property on="ArmRotateV" class="WFChart (strict)"("History Data"=dbl[] []) -> (error out=w285:errorcluster)  [unwired: 2 in, 1 out]
          n152 = property on="ArmExtensionV" class="WFChart (strict)"("History Data"=dbl[] []) -> (error out=w287:errorcluster)  [unwired: 2 in, 1 out]
        }
      }
      n153 = Merge Errors(w198, w197, w196, w195) -> (w194:errorcluster)
      n154 = feedback-in #7(w194) -> ()
      n155 = call-poly <vilib>:"CTRE_Phoenix_MotorController_Get_Enhanced.vi"("PhoenixMotorControlDevRef"=w237, "error in"=w236) -> ("Output Voltage"=w259:dbl)  [unwired: 9 in, 4 out]
      n156 = call-poly <vilib>:"CTRE_Phoenix_MotorController_Get_Enhanced.vi"("PhoenixMotorControlDevRef"=w235, "error in"=w234) -> ("Output Voltage"=w260:dbl)  [unwired: 9 in, 4 out]
      n157 = call <vilib>:"CTRE_Phoenix_MotorControl_GetMotionProfileStatus.vi"("error in"=w236, "PhoenixMotorControlDevRef"=w237) -> ("Motion Profile Status"=w254:T10)  [unwired: 7 in, 2 out]
      n158 = call <vilib>:"CTRE_Phoenix_MotorControl_GetActiveTrajectory.vi"("PhoenixMotorControlDevRef"=w237, "error in"=w236) -> ("Position (Sensor Units)"=w280:i32, "Velocity (Sensor Units per 100 ms)"=w279:i32)  [unwired: 9 in, 3 out]
      n159 = call-poly <vilib>:"CTRE_Phoenix_MotorController_Get_Enhanced.vi"("PhoenixMotorControlDevRef"=w237, "error in"=w236) -> ("Position (Raw Sensor Units)"=w278:i32, "Velocity (Raw Sensor Units per 100 ms)"=w262:i32)  [unwired: 10 in, 2 out]
      n160 = call <vilib>:"CTRE_Phoenix_MotorControl_GetMotionProfileStatus.vi"("error in"=w234, "PhoenixMotorControlDevRef"=w235) -> ("Motion Profile Status"=w255:T10)  [unwired: 7 in, 2 out]
      n161 = call <vilib>:"CTRE_Phoenix_MotorControl_GetActiveTrajectory.vi"("PhoenixMotorControlDevRef"=w235, "error in"=w234) -> ("Position (Sensor Units)"=w277:i32, "Velocity (Sensor Units per 100 ms)"=w276:i32)  [unwired: 9 in, 3 out]
      n162 = call-poly <vilib>:"CTRE_Phoenix_MotorController_Get_Enhanced.vi"("PhoenixMotorControlDevRef"=w235, "error in"=w234) -> ("Position (Raw Sensor Units)"=w275:i32, "Velocity (Raw Sensor Units per 100 ms)"=w265:i32)  [unwired: 10 in, 2 out]
      n163 = Unbundle By Name(w255) -> ("Output Enable"=w268:i32, "Is Last?"=w231:bool)
      n164 = Unbundle By Name(w254) -> ("Output Enable"=w274:i32, "Is Last?"=w230:bool)
      n165 = Multiply(x=w262, y=10) -> (x*y=w263:i32)
      n166 = Multiply(x=w265, y=10) -> (x*y=w266:i32)
      n167 = Bundle("Position (Sensor Units)"=w280, "Velocity (Sensor Units per 100 ms)"=w279, "Position (Raw Sensor Units)"=w278, w263) -> (w229:T19)  [unwired: 1 in]
      n168 = Bundle("Position (Sensor Units)"=w277, "Velocity (Sensor Units per 100 ms)"=w276, "Position (Raw Sensor Units)"=w275, w266) -> (w228:T19)  [unwired: 1 in]
      n169 = Equal?(x=1, y=w274) -> (x = y?=w272:bool)
      n170 = Equal?(x=1, y=w268) -> (x = y?=w270:bool)
      n171 = Compound Arithmetic op=AND(w231, w230) -> (w202:bool)
      n172 = Unbundle(w229) -> ("Position (Sensor Units)"=w227:i32, "Position (Raw Sensor Units)"=w226:i32)  [unwired: 2 out]
      n173 = Unbundle(w228) -> ("Position (Sensor Units)"=w225:i32, "Position (Raw Sensor Units)"=w224:i32)  [unwired: 2 out]
      n174 = Compound Arithmetic op=AND(w272, invert w230) -> (w271:bool)
      n175 = Compound Arithmetic op=AND(w270, invert w231) -> (w267:bool)
      n176 = call "EdgeDetector.vi"("DetectorType"=EdgeDetector_Type."RisingEdge", "Input"=w202) -> ("Edge"=w200:bool)
      n177 = Subtract(x=w225, y=w224) -> (x-y=w232:i32)
      n178 = Subtract(x=w227, y=w226) -> (x-y=w233:i32)
      n179 = Absolute Value(x=w232) -> (abs(x)=w218:i32)
      n180 = Absolute Value(x=w233) -> (abs(x)=w220:i32)
      n181 = Divide(x=w220, y=w219) -> (x/y=w253:dbl)
      n182 = Divide(x=w218, y=w217) -> (x/y=w252:dbl)
      n183 = Greater?(x=w253, y=w250) -> (0:w249:bool)
      n184 = Greater?(x=w252, y=w251) -> (0:w248:bool)
      n185 = case shown="True" w200 {
        selector: w200 -> [_ w283]
        tunnel: "ArmCompleteNotifier" -> [_ w282]
        frame False {
        }
        frame True {
          n186 = Send Notification(notification=w283, notifier=w282) -> ()  [unwired: 1 in, 2 out]
        }
      }
      n187 = call "Timed_DeBounce.vi"("Input"=w249, "Reset"=w209, "Hold Time(ms)"=w247) -> ("Output"=w246:bool)
      n188 = call "Timed_DeBounce.vi"("Input"=w248, "Reset"=w209, "Hold Time(ms)"=w247) -> ("Output"=w245:bool)
      n189 = feedback #8() -> (w256:T3)  [unwired: 1 in]
      n190 = Select(t=MotionProfileControlState."Auto_Run" ("Arm Control State"), s=w209, f=w256) -> (s? t:f=w257:T3)
      n191 = Select(t=MotionProfileControlState."Auto_Idle" ("Arm Control State"), s=w202, f=w257) -> (s? t:f=w243:T3)
      n192 = Or(x=w246, y=w245) -> (x .or. y?=w223:bool)
      n193 = And(x=w223, y=w221) -> (x .and. y?=w222:bool)
      n194 = Select(t=MotionProfileControlState."Manual", s=w222, f=w243) -> (s? t:f=w244:T3)
      n195 = feedback-in #8(w244) -> ()
      "MP Send State" <- w203
    }
  }
  "Arm Control State" <- w24
  "Extension" <- w76
  "Rotate" <- w75
  "Rotate" <- w54
  "Extension" <- w53
  n196 = feedback-in #2(w24) -> ()
  n197 = Build Array(WPI_DriverStationRobotMode2."Teleop Enabled" ("Robot Mode"), WPI_DriverStationRobotMode2."Autonomous Enabled" ("Robot Mode")) -> (w30:T13[])
  n198 = call <vilib>:"WPI_DriverStationGetModeAndStatus.vi"() -> ("Robot Mode"=w34:T13)  [unwired: 10 in, 1 out]
  n199 = Equal?(x=w30, y=w34) -> (x = y?=w33:bool[])
  n200 = Unbundle By Name(w75) -> ("Velocity (Sensor Units per 100 ms)"=w57:i32, "Position (Raw Sensor Units)"=w90:i32)
  n201 = Unbundle By Name(w76) -> ("Velocity (Sensor Units per 100 ms)"=w60:i32, "Position (Raw Sensor Units)"=w91:i32)
  n202 = Or Array Elements(Boolean array=w33) -> (logical OR=w29:bool)
  n203 = And(x=w29, y=w96) -> (x .and. y?=w51:bool)
  n204 = And(x=w29, y=w98) -> (x .and. y?=w50:bool)
  n205 = Divide(x=w91, y="extend sensor unit coversion (ticks/in)") -> (x/y=w89:dbl)
  n206 = Divide(x=w90, y="rotate sensor unit conversion (ticks/rad)") -> (x/y=w88:dbl)
  n207 = call "CoordinateConvert_ArmToCartesian.vi"("Radius (in)"=w89, "Angle (rad)"=w88) -> ("Y (in)"=w19:dbl, "X (in)"=w20:dbl)
  n208 = call "HistoricMaxMagnitude.vi"("Reset"="Reset Extend Max", "Value"=w60) -> ("Max"=→"Max Extend Speed (Sensor Units per 100 ms)":dbl)
  n209 = call "HistoricMaxMagnitude.vi"("Reset"="Reset Rotate Max", "Value"=w57) -> ("Max"=→"Max Rotate Speed (Sensor Units per 100 ms)":dbl)
  n210 = case shown="True" w51 {
    tunnel: w76 -> [_ w462]
    tunnel: w94 -> [_ w461]
    frame False {
    }
    frame True {
      "ArmExtension" <- w462
      "ArmExtensionV" <- w461
    }
  }
  n211 = case shown="True" w50 {
    tunnel: w75 -> [_ w464]
    tunnel: w95 -> [_ w463]
    frame False {
    }
    frame True {
      "ArmRotation" <- w464
      "ArmRotateV" <- w463
    }
  }
  n212 = Or(x=w51, y=w50) -> (x .or. y?=w47:bool)
  n213 = call "EdgeDetector.vi"("DetectorType"=EdgeDetector_Type."RisingEdge", "Input"=w47) -> ("Edge"=w35:bool)
  n214 = global write "LEDData.vi" "ArmHeight"(w19) -> ()
  n215 = feedback #9() -> (w45:dbl[])  [unwired: 1 in]
  n216 = Select(t=w40, s=w35, f=w45) -> (s? t:f=w44:dbl[])
  n217 = feedback #10() -> (w36:cluster{dbl[], dbl[]})  [unwired: 1 in]
  n218 = case shown="True" w35 {
    tunnel: "Arm Extend Motion Profile" -> [_ w470]
    tunnel: "Arm Rotate Motion Profile" -> [_ w469]
    tunnel: [w465 w466] -> w37
    tunnel: w36 -> [w465 _]
    frame False {
    }
    frame True {
      n219 = for {
        tunnel: w470 -> [w476] mode=indexing
        tunnel: w469 -> [w475] mode=indexing
        tunnel: [w472] -> w468 mode=indexing
        tunnel: [w471] -> w467 mode=indexing
        n220 = Unbundle By Name(w476) -> ("Position"=w474:dbl)
        n221 = Unbundle By Name(w475) -> ("Position"=w473:dbl)
        n222 = call "CoordinateConvert_ArmToCartesian.vi"("Radius (in)"=w474, "Angle (rad)"=w473) -> ("Y (in)"=w471:dbl, "X (in)"=w472:dbl)
      }
      n223 = Bundle(w468, w467) -> (w466:cluster{dbl[], dbl[]})  [unwired: 1 in]
    }
  }
  n224 = feedback-in #10(w37) -> ()
  n225 = feedback #11() -> (w41:dbl[])  [unwired: 1 in]
  n226 = Select(t=w40, s=w35, f=w41) -> (s? t:f=w43:dbl[])
  n227 = case shown="False" w47 {
    tunnel: w20 -> [_ w484]
    tunnel: w19 -> [_ w483]
    tunnel: [w477 w482] -> w48
    tunnel: [w478 w481] -> w42
    tunnel: w44 -> [w477 w480]
    tunnel: w43 -> [w478 w479]
    frame False {
    }
    frame True {
      n228 = Build Array (concatenate)(w479, w484) -> (w481:dbl[])
      n229 = Build Array (concatenate)(w480, w483) -> (w482:dbl[])
    }
  }
  n230 = feedback-in #9(w48) -> ()
  n231 = feedback-in #11(w42) -> ()
  n232 = Build Array(w74, w20) -> (w87:dbl[])
  n233 = Build Array(w74, w19) -> (w86:dbl[])
  n234 = call "SetArmPosition.vi"("ArmYPosition"=w19, "ArmXPosition"=w20) -> ()  [unwired: 1 in]
  n235 = Bundle("t"=w42, "t"=w48) -> (w49:cluster{"t":dbl[], "t":dbl[]})  [unwired: 1 in]
  n236 = Bundle(w87, w86) -> (w85:cluster{dbl[], dbl[]})  [unwired: 1 in]
  n237 = Build Array(w37, w49, w85) -> (→"Arm Tracking":cluster{"t":dbl[], "t":dbl[]}[])
